vi "testRun.vi"() -> ()   [LabVIEW 2025, in "HydraulicTest.lvclass"]
uses:
  HydraulicTest.lvclass
  H1 Hydraulic.lvclass
  <vilib>/measure/NI_MABase.lvlib
panel:
  in  "loop":u32=50
  # "Not exceed 50 ms"
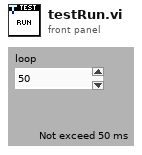
[diagram p1: front panel]
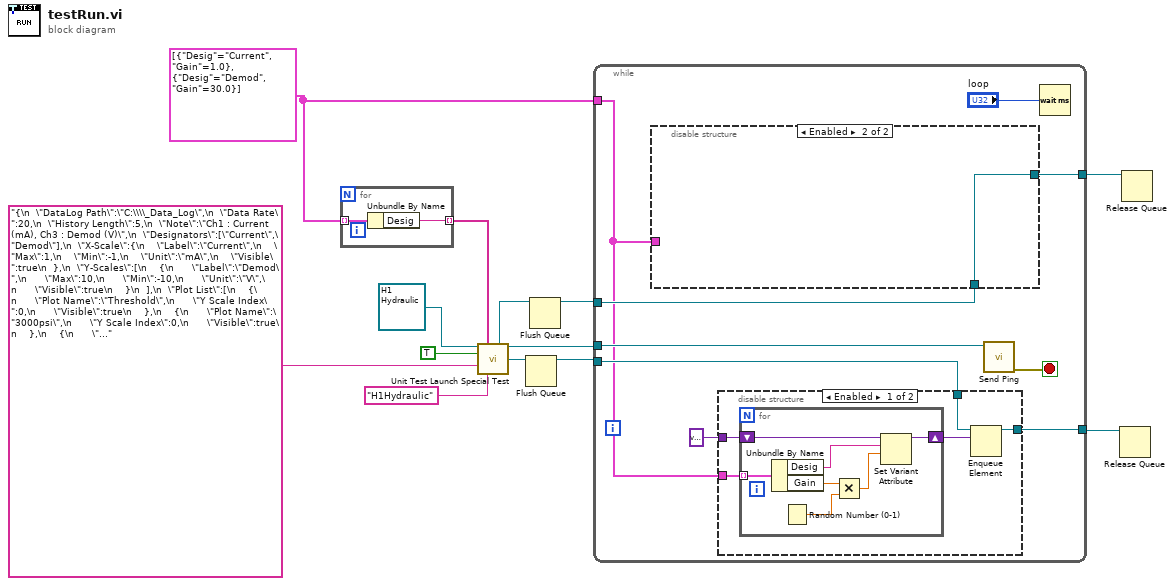
[diagram p0: block diagram]
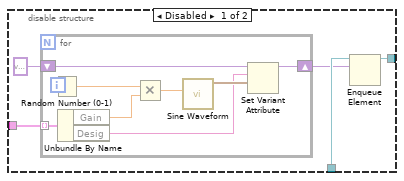
[diagram p2: hidden frame]
diagram:
  w1 = cluster{"Desig":string, "Gain":dbl}[] [{"Desig"="Current", "Gain"=1.0}, {"Desig"="Demod", "Gain"=30.0}] ("Sim Param")
  n1 = for {
    tunnel: w1 -> [w15] mode=indexing
    tunnel: [w14] -> w10 mode=indexing
    n2 = Unbundle By Name(w15) -> ("Desig"=w14:string)
  }
  n3 = call "Unit Test Launch Special Test.vi"("Special Test Class"=refnum<class "H1 Hydraulic.lvclass"> refnum ("Sensitivity.lvlib:Sensitivity.lvclass"), "Subscription Alias"=w10, "Auto Launched"=TRUE, "<JSON>"="{\n  \"DataLog Path\":\"C:\\\\_Data_Log\",\n  \"Data Rate\":20,\n  \"History Length\":5,\n  \"Note\":\"Ch1 : Current (mA), Ch3 : Demod (V)\",\n  \"Designators\":[\"Current\",\"Demod\"],\n  \"X-Scale\":{\n    \"Label\":\"Current\",\n    \"Max\":1,\n    \"Min\":-1,\n    \"Unit\":\"mA\",\n    \"Visible\":true\n  },\n  \"Y-Scales\":[\n    {\n      \"Label\":\"Demod\",\n      \"Max\":10,\n      \"Min\":-10,\n      \"Unit\":\"V\",\n      \"Visible\":true\n    }\n  ],\n  \"Plot List\":[\n    {\n      \"Plot Name\":\"Threshold\",\n      \"Y Scale Index\":0,\n      \"Visible\":true\n    },\n    {\n      \"Plot Name\":\"3000psi\",\n      \"Y Scale Index\":0,\n      \"Visible\":true\n    },\n    {\n      \"Plot Name\":\"1500psi\",\n      \"Y Scale Index\":0,\n      \"Visible\":true\n    },\n    {\n      \"Plot Name\":\"140psi\",\n      \"Y Scale Index\":0,\n      \"Visible\":true\n    }\n]\n}" ("Settings_JSON_"), "Debug Alias"="H1Hydraulic") -> ("Data Queue out"=w4:refnum<queue>, "ST Enqueuer out"=w3:refnum<class "Message Enqueuer.lvclass">, "Fast Map Queue out"=w2:refnum<queue>)  [unwired: 2 in, 6 out]
  n4 = Flush Queue(queue=w2) -> (queue out=w8:refnum<queue>)  [unwired: 1 in, 2 out]
  n5 = Flush Queue(queue=w4) -> (queue out=w7:refnum<queue>)  [unwired: 1 in, 2 out]
  n6 = while {
    tunnel: w3 -> [w24]
    tunnel: w8 -> [w21]
    tunnel: [w19] -> w6
    tunnel: w1 -> [w18]
    tunnel: w7 -> [w23]
    tunnel: [w20] -> w5
    stop <- w17 stop-if-true
    n7 = disable-structure shown="Enabled" {
      disable-tunnel: w23 -> [w28 w38]
      disable-tunnel: [w27 w38] -> w19
      disable-tunnel: w18 -> [w26 _]
      frame Disabled {
        n8 = for {
          shift-right: [w36] -> w25
          shift-left: variant ("variant") -> [w37]
          tunnel: w26 -> [w34] mode=indexing
          n9 = Random Number (0-1)() -> (number: 0 to 1=w30:dbl)
          n10 = Unbundle By Name(w34) -> ("Gain"=w32:dbl, "Desig"=w33:string)
          n11 = Multiply(x=w30, y=w32) -> (x*y=w31:dbl)
          n12 = call <vilib>:"Sine Waveform.vi"("amplitude"=w31) -> ("signal out"=w35:waveform(dbl))  [unwired: 9 in, 1 out]
          n13 = Set Variant Attribute(Variant=w37, name=w33, value=w35) -> (Variant out=w36:variant)  [unwired: 1 in, 2 out]
        }
        n14 = Enqueue Element(queue=w28, element=w25) -> (queue out=w27:refnum<queue>)  [unwired: 2 in, 2 out]
      }
      frame Enabled {
      }
    }
    n15 = disable-structure shown="Enabled" {
      disable-tunnel: variant ("variant") -> [w43 _]
      disable-tunnel: w21 -> [w42 w51]
      disable-tunnel: [w41 w51] -> w20
      disable-tunnel: w18 -> [w40 _]
      frame Enabled {
        n16 = for {
          shift-right: [w49] -> w39
          shift-left: w43 -> [w50]
          tunnel: w40 -> [w48] mode=indexing
          n17 = Unbundle By Name(w48) -> ("Desig"=w47:string, "Gain"=w46:dbl)
          n18 = Random Number (0-1)() -> (number: 0 to 1=w45:dbl)
          n19 = Multiply(x=w46, y=w45) -> (x*y=w44:dbl)
          n20 = Set Variant Attribute(Variant=w50, name=w47, value=w44) -> (Variant out=w49:variant)  [unwired: 1 in, 2 out]
        }
        n21 = Enqueue Element(queue=w42, element=w39) -> (queue out=w41:refnum<queue>)  [unwired: 2 in, 2 out]
      }
      frame Disabled {
      }
    }
    n22 = call "Send Ping.vi"("Message Enqueuer"=w24) -> ("error out"=w17:errorcluster)  [unwired: 6 in, 4 out]
    n23 = Wait (ms)(milliseconds to wait="loop") -> ()  [unwired: 1 out]
  }
  n24 = Release Queue(queue=w5) -> ()  [unwired: 2 in, 3 out]
  n25 = Release Queue(queue=w6) -> ()  [unwired: 2 in, 3 out]
